vi "Destroy User Event - Stop.vi"(8 "error in (no error)":errorcluster, 11 "User events":T1) -> (0 "error out":errorcluster)   [LabVIEW 2020, in "oled User Event - Stop.lvlib"]
doc: "Destroy the user event, even if there is an incoming error."
uses:
  oled User Event - Stop.lvlib
  controls/HL Acq Data.ctl
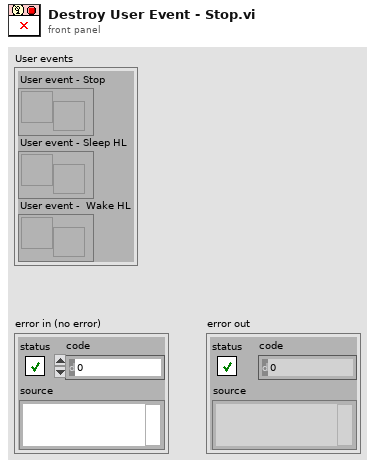
[diagram p1: front panel]
types:
  T1 = cluster{"User event - Stop":refnum<user-event>, "User event - Sleep HL":refnum<user-event>, "User event -  Wake HL":refnum<user-event>}
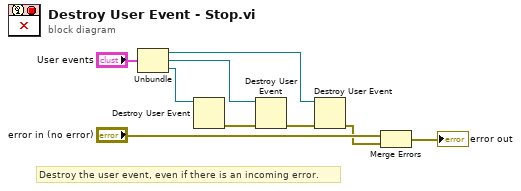
[diagram p0: block diagram]
diagram:
  # "Destroy the user event, even if there is an incoming error."
  n1 = Unbundle("User events") -> ("User event - Stop"=w2:refnum<user-event>, "User event - Sleep HL"=w3:refnum<user-event>, "User event -  Wake HL"=w7:refnum<user-event>)
  n2 = Destroy User Event(user event=w7) -> (error out=w6:errorcluster)  [unwired: 1 in]
  n3 = Destroy User Event(user event=w3, error in=w6) -> (error out=w5:errorcluster)
  n4 = Destroy User Event(user event=w2, error in=w5) -> (error out=w4:errorcluster)
  n5 = Merge Errors("error in (no error)", w4) -> (→"error out":errorcluster)
